vi "CollectAndFormatResult.vi"(7 "Mode":T1, 9 "Param/Result":T2, 10 "Count":u8) -> (3 "Read Data":string)   [LabVIEW 2025]
uses:
  FormatData_ctl.ctl
  Mode_ctl.ctl
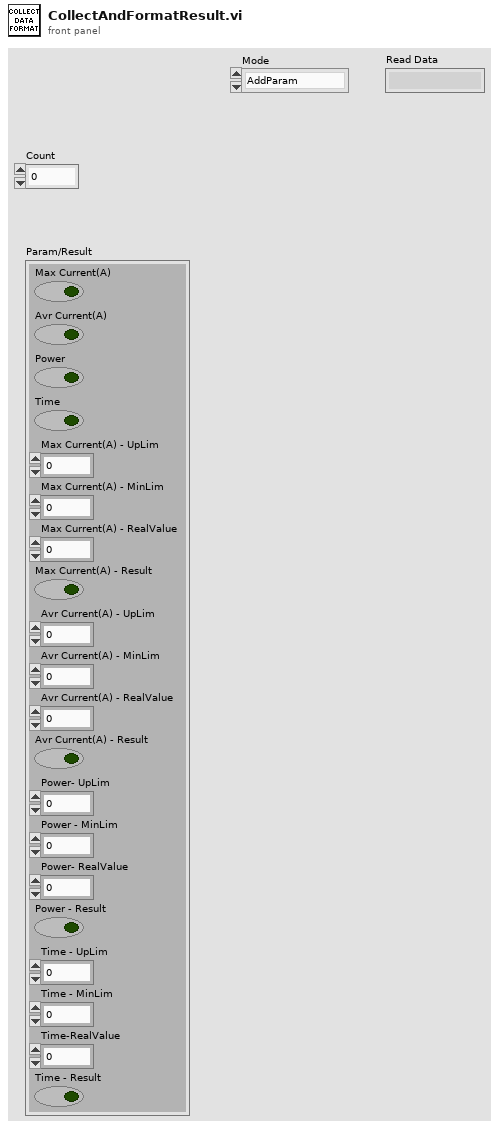
[diagram p1: front panel]
types:
  T1 = typedef "Mode_ctl.ctl" = enum16{"AddParam", "AddResult", "ReadData", "Clear"}
  T2 = typedef "FormatData_ctl.ctl" = cluster{"Max Current(A)":bool, "Avr Current(A)":bool, "Power":bool, "Time":bool, "Max Current(A) - UpLim":dbl, "Max Current(A) - MinLim":dbl, "Max Current(A) - RealValue":dbl, "Max Current(A) - Result":bool, "Avr Current(A) - UpLim":dbl, "Avr Current(A) - MinLim":dbl, "Avr Current(A) - RealValue":dbl, "Avr Current(A) - Result":bool, "Power- UpLim":dbl, "Power - MinLim":dbl, "Power- RealValue":dbl, "Power - Result":bool, "Time - UpLim":dbl, "Time - MinLim":dbl, "Time-RealValue":dbl, "Time - Result":bool}
  T3 = cluster{"Max Current(A)":bool, "Max Current(A) - MinLim":dbl, "Max Current(A) - UpLim":dbl, "Max Current(A) - RealValue":dbl, "Max Current(A) - Result":bool}
  T4 = cluster{"Avr Current(A)":bool, "Avr Current(A) - MinLim":dbl, "Avr Current(A) - UpLim":dbl, "Avr Current(A) - RealValue":dbl, "Avr Current(A) - Result":bool}
  T5 = cluster{"Power":bool, "Power - MinLim":dbl, "Power- UpLim":dbl, "Power- RealValue":dbl, "Power - Result":bool}
  T6 = cluster{"Time":bool, "Time - MinLim":dbl, "Time - UpLim":dbl, "Time-RealValue":dbl, "Time - Result":bool}
  T7 = cluster{"Time":bool, "Time - MinLim":dbl, "Time - UpLim":dbl, "Time-RealValue":dbl, "Time - Result":bool}[]
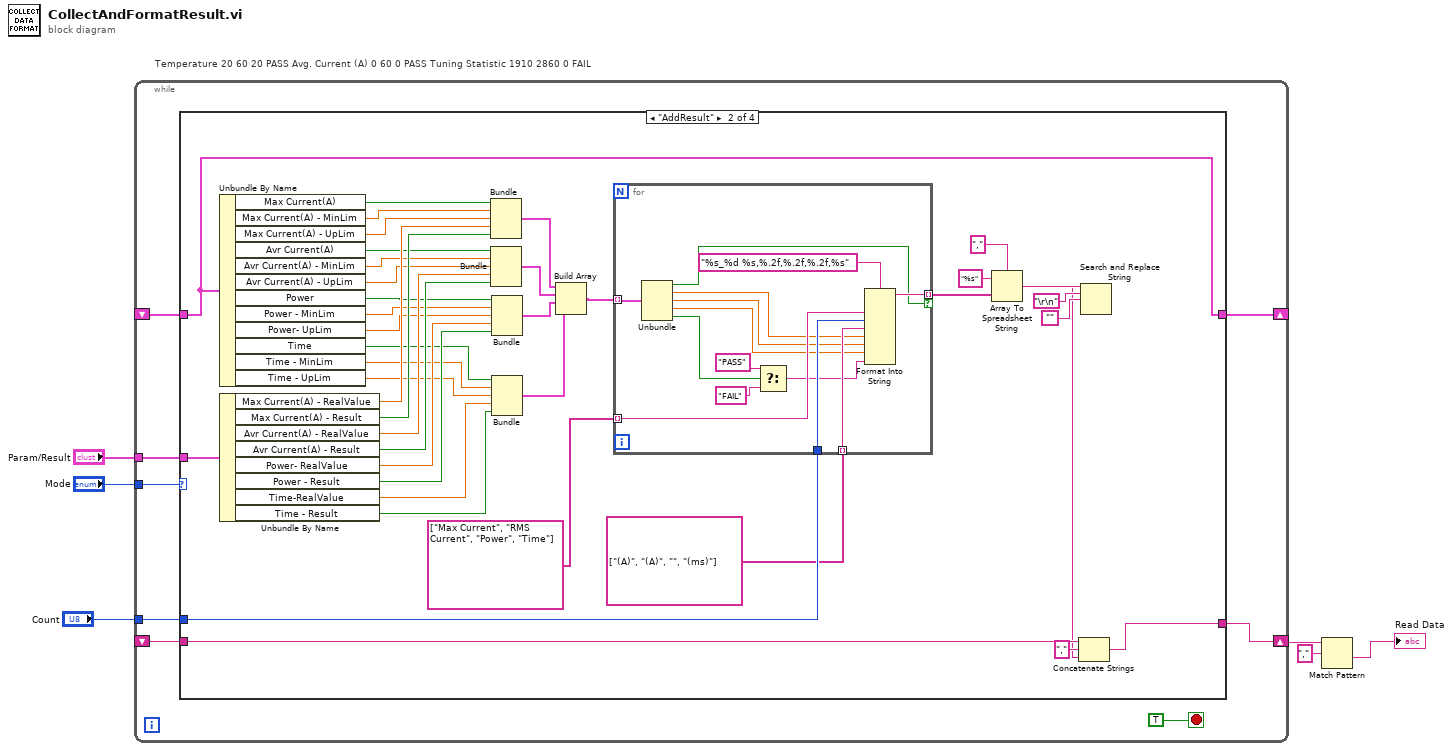
[diagram p0: block diagram]
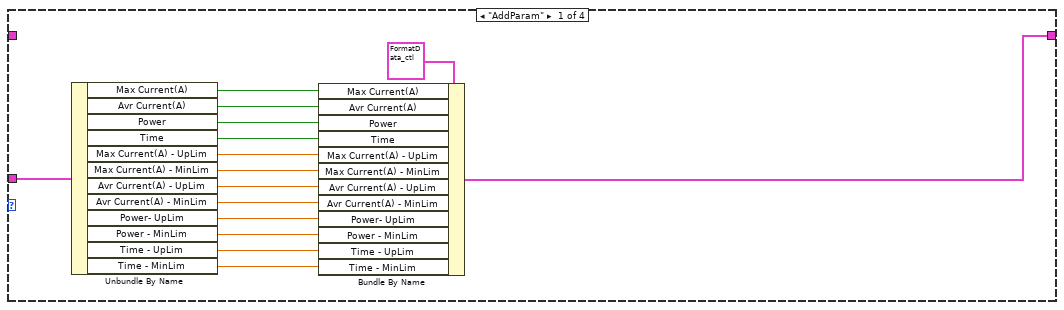
[diagram p2: hidden frame]
diagram:
  # "Temperature\t20\t60\t20\tPASS\tAvg. Current (A)\t0\t60\t0\tPASS\tTuning Statistic\t1910\t2860\t0\tFAIL"
  n1 = while {
    tunnel: "Mode" -> [w13]
    tunnel: "Param/Result" -> [w12]
    shift-right: [w11] -> _
    shift-left: _ -> [w10]
    tunnel: "Count" -> [w9]
    shift-right: [w8] -> w3
    shift-left: _ -> [w7]
    stop <- TRUE stop-if-true
    n2 = case shown="\"AddResult\"" w13 {
      tunnel: w12 -> [w29 w69 _ _]
      tunnel: [w15 w38 w85 _] -> w11
      tunnel: w10 -> [_ w38 w85 _]
      tunnel: w9 -> [_ w42 _ _]
      tunnel: [_ w37 w84 _] -> w8
      tunnel: w7 -> [_ w32 w84 _]
      frame "AddParam" {
        n3 = Unbundle By Name(w29) -> ("Max Current(A)"=w28:bool, "Avr Current(A)"=w27:bool, "Power"=w26:bool, "Time"=w25:bool, "Max Current(A) - UpLim"=w24:dbl, "Max Current(A) - MinLim"=w23:dbl, "Avr Current(A) - UpLim"=w22:dbl, "Avr Current(A) - MinLim"=w21:dbl, "Power- UpLim"=w20:dbl, "Power - MinLim"=w19:dbl, "Time - UpLim"=w18:dbl, "Time - MinLim"=w17:dbl)
        n4 = Bundle By Name(cluster=T2 {"Max Current(A)"=FALSE, "Avr Current(A)"=FALSE, "Power"=FALSE, "Time"=FALSE, "Max Current(A) - UpLim"=0.0, "Max Current(A) - MinLim"=0.0, "Max Current(A) - RealValue"=0.0, "Max Current(A) - Result"=FALSE, "Avr Current(A) - UpLim"=0.0, "Avr Current(A) - MinLim"=0.0, "Avr Current(A) - RealValue"=0.0, "Avr Current(A) - Result"=FALSE, "Power- UpLim"=0.0, "Power - MinLim"=0.0, "Power- RealValue"=0.0, "Power - Result"=FALSE, "Time - UpLim"=0.0, "Time - MinLim"=0.0, "Time-RealValue"=0.0, "Time - Result"=FALSE}, "Max Current(A)"=w28, "Avr Current(A)"=w27, "Power"=w26, "Time"=w25, "Max Current(A) - UpLim"=w24, "Max Current(A) - MinLim"=w23, "Avr Current(A) - UpLim"=w22, "Avr Current(A) - MinLim"=w21, "Power- UpLim"=w20, "Power - MinLim"=w19, "Time - UpLim"=w18, "Time - MinLim"=w17) -> (w15:T2)
      }
      frame "AddResult" {
        n5 = Unbundle By Name(w38) -> ("Max Current(A)"=w68:bool, "Max Current(A) - MinLim"=w67:dbl, "Max Current(A) - UpLim"=w66:dbl, "Avr Current(A)"=w63:bool, "Avr Current(A) - MinLim"=w62:dbl, "Avr Current(A) - UpLim"=w61:dbl, "Power"=w58:bool, "Power - MinLim"=w57:dbl, "Power- UpLim"=w56:dbl, "Time"=w53:bool, "Time - MinLim"=w52:dbl, "Time - UpLim"=w51:dbl)
        n6 = Unbundle By Name(w69) -> ("Max Current(A) - RealValue"=w65:dbl, "Max Current(A) - Result"=w64:bool, "Avr Current(A) - RealValue"=w60:dbl, "Avr Current(A) - Result"=w59:bool, "Power- RealValue"=w55:dbl, "Power - Result"=w54:bool, "Time-RealValue"=w50:dbl, "Time - Result"=w49:bool)
        n7 = Bundle("Max Current(A)"=w68, "Max Current(A) - MinLim"=w67, "Max Current(A) - UpLim"=w66, "Max Current(A) - RealValue"=w65, "Max Current(A) - Result"=w64) -> (w48:T3)  [unwired: 1 in]
        n8 = Bundle("Avr Current(A)"=w63, "Avr Current(A) - MinLim"=w62, "Avr Current(A) - UpLim"=w61, "Avr Current(A) - RealValue"=w60, "Avr Current(A) - Result"=w59) -> (w47:T4)  [unwired: 1 in]
        n9 = Bundle("Power"=w58, "Power - MinLim"=w57, "Power- UpLim"=w56, "Power- RealValue"=w55, "Power - Result"=w54) -> (w46:T5)  [unwired: 1 in]
        n10 = Bundle("Time"=w53, "Time - MinLim"=w52, "Time - UpLim"=w51, "Time-RealValue"=w50, "Time - Result"=w49) -> (w45:T6)  [unwired: 1 in]
        n11 = Build Array(w48, w47, w46, w45) -> (w44:T7)
        n12 = for {
          tunnel: w44 -> [w83] mode=indexing
          tunnel: string[] ["Max Current", "RMS Current", "Power", "Time"] ("行首字符串[]") -> [w76] mode=indexing
          tunnel: w42 -> [w75]
          tunnel: [w81] -> w41 mode=indexing if=w80
          tunnel: string[] ["(A)", "(A)", "", "(ms)"] ("行首字符串[]") -> [w74] mode=indexing
          n13 = Unbundle(w83) -> ("Time"=w80:bool, "Time - MinLim"=w73:dbl, "Time - UpLim"=w72:dbl, "Time-RealValue"=w71:dbl, "Time - Result"=w79:bool)
          n14 = Select(t="PASS", s=w79, f="FAIL") -> (s? t:f=w70:string)
          n15 = Format Into String(format string="%s_%d %s,%.2f,%.2f,%.2f,%s", w76, w75, w74, w73, w72, w71, w70) -> (resulting string=w81:string)  [unwired: 2 in, 1 out]
        }
        n16 = Array To Spreadsheet String(delimiter (Tab)=",", array=w41, 3:"%s" ("format string")) -> (spreadsheet string=w36:string)
        n17 = Search and Replace String(input string=w36, search string="\r\n", replace string="") -> (result string=w31:string)  [unwired: 5 in, 3 out]
        n18 = Concatenate Strings(w32, "," ("string"), w31) -> (w37:string)
      }
      frame "ReadData" {
      }
      frame "Clear" {
      }
    }
  }
  n19 = Match Pattern(string=w3, regular expression=",") -> (after substring=→"Read Data":string)  [unwired: 1 in, 3 out]
